vi "Initialize Reader Data.vi"(8 "error in (no error)":errorcluster, 11 "CIF_Iceoryx_BB in":refnum<class "CIF_Iceoryx_BB.lvclass">) -> (0 "error out":errorcluster, 3 "CIF_Iceoryx_BB out":refnum<class "CIF_Iceoryx_BB.lvclass">)   [LabVIEW 2021, in "CIF_Iceoryx_BB.lvclass"]
uses:
  CIF_Iceoryx_BB.lvclass
  CIF_Iceoryx_BB.lvclass/CIF_Iceoryx_BB.ctl
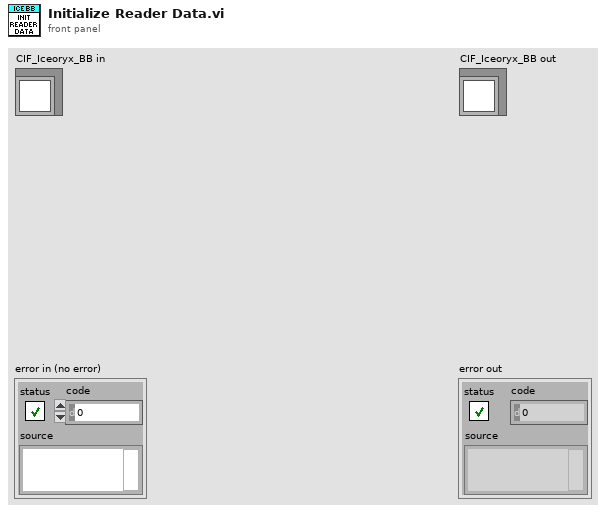
[diagram p1: front panel]
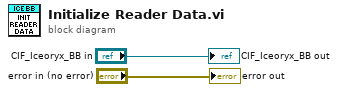
[diagram p0: block diagram]
diagram:
  "error out" <- "error in (no error)"
  "CIF_Iceoryx_BB out" <- "CIF_Iceoryx_BB in"
